vi "[ce] Create menu at runtime.vi"(4 "enable tracking (T)":bool=TRUE, 6 "after item tag":string, 7 "menu tag":string, 8 "error in":errorcluster, 9 "operation (replace)":T1(ring)=enum."replace existing menu", 10 "menu descriptor":string, 11 "menu":refnum<k9>) -> (0 "error out":errorcluster, 3 "dup menu":refnum<k9>)   [LabVIEW 2021]
doc: "The VI takes a menu descriptor and creates new menu on base of it. It can also insert or replace submenu(s) in an existing menu.\n\n<B>menu tag</B> specifies a submenu where new submenu(s) are inserted. An empty string specifies menubar. \n\n<B>after item tag</B> specifies the position where new submenu(s) are inserted. It is only used if <B>operation</B> is <insert into existing menu>. An empty string specifies the beginning of the existing submenu.\n\n<B>operation</B> specifies one of the following operations:\n <insert into existing menu> inserts the new submenu(s) to <B>menu tag</B> submenu at <B>after item tag</B> position.\n <append to existing submenu> appends the new submenu(s) to the end of <B>menu tag</B> submenu.\n <replace existing menu> replaces all the items in the <B>menu tag</B> submenu with the new submenu(s).\n\n<B>menu descriptor</B> is a multi-line string where each line contains a menu item attributes. Empty lines and lines beginning with semicolon (;) are ignored. A line starting with a dash sign (-) forms a separator in menu. A descriptor line has the following format:\n\n [SubMenuSign] ItemName : ItemTag [ : ItemParams [ : comments] ]\n\nSybMenuSign is optional parameter that can be either greater-than sign (>) marking the beginning of new submenu or less-than sign (<) marking the end of submenu. If a line begins with less-than sign (<), the rest of the line is ignored. You can form nested submenus providing that each '>' block is terminated with '<'.\n\nItemName and ItemTag are respectively a name of menu item and a tag of menu item. If an item name includes a underscore sign (_), the following character is used for ALT navigation. \n\nItemParams can contain optional specificators of the menu item separated by spaces. The specificators are not case-sensitive. You can use the following specificators:\nDIS - menu item is disabled\nCHK - menu item is checked\nKEY=CHAR - specifies a shortcut keys combination. If CHAR begins with '@' sign, the shortcut is CTRL-SHIFT-CHAR; otherwise, it is CTRL-CHAR.\n\n<B>Example:</B>\n------------\n; File menu\n> File : file\n _Open... : open : key=O\n _Close... : close : key=C\n - ;separator\n ; nested submenu\n > Configuration : config\n Parameter 1 : cfg_1 : CHK : checked\n Parameter 2 : cfg_2 : DIS : disabled\n <\n - ;separator\n E_xit : exit : key=X\n<\n; Mode menu\n> Mode : mode\nmode 1 : mode1 : KEY=@A CHK\nmode 2 : mode2 : KEY=@B DIS\nmode 3 : mode3 : KEY=@C\n<\n\n::: CalcExpress Toolkit :::\nCopyright (c) 2000-2026 Konstantin Shifershteyn. All rights reserved."
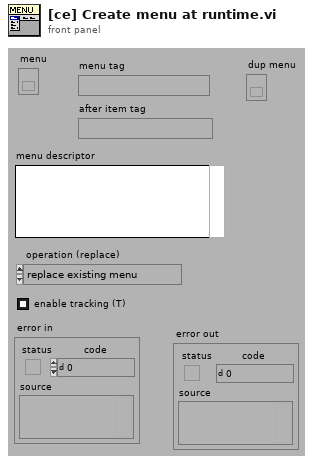
[diagram p1: front panel]
types:
  T1 = enum16{"insert into existing menu", "append to existing menu", "replace existing menu"}
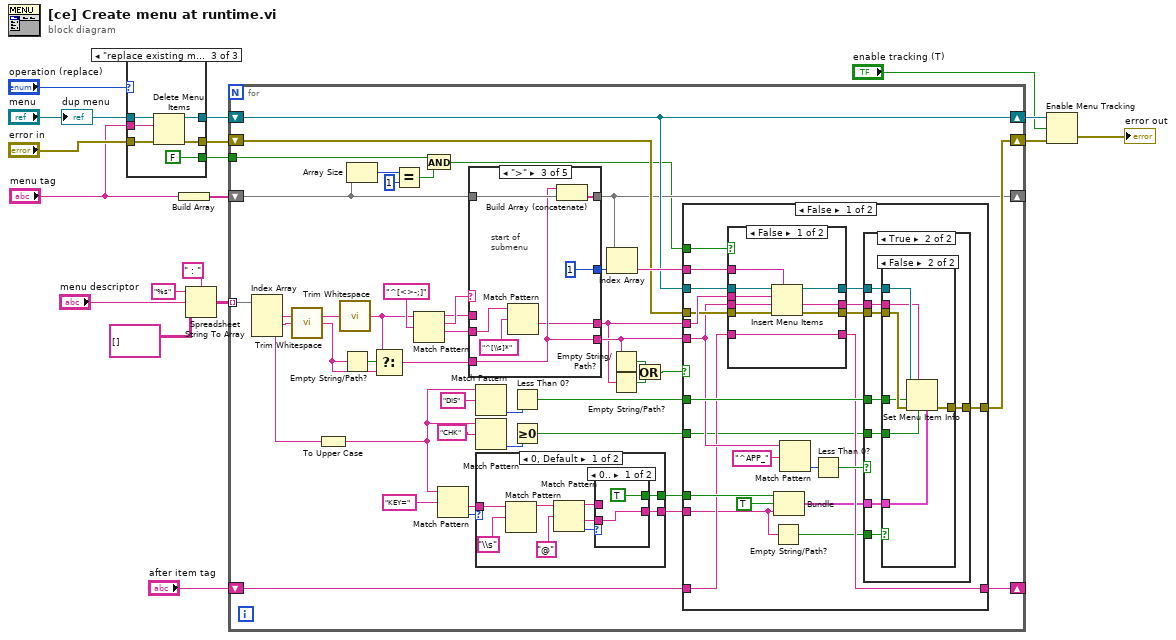
[diagram p0: block diagram]
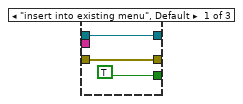
[diagram p2: hidden frame]
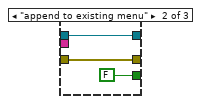
[diagram p3: hidden frame]
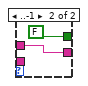
[diagram p4: hidden frame]
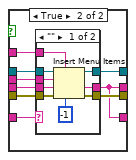
[diagram p6: hidden frame]
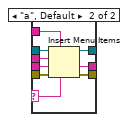
[diagram p7: hidden frame]
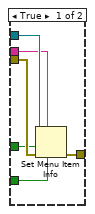
[diagram p9: hidden frame]
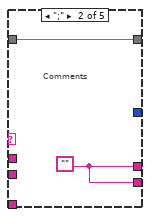
[diagram p12: hidden frame]
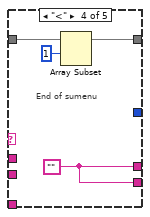
[diagram p13: hidden frame]
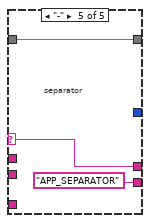
[diagram p14: hidden frame]
diagram:
  n1 = case shown="\"replace existing menu\"" "operation (replace)" {
    tunnel: [w21 w24 w30] -> w14
    tunnel: "menu" -> [w21 w24 w29]
    tunnel: [w20 w23 w28] -> w13
    tunnel: "error in" -> [w20 w23 w27]
    tunnel: [TRUE FALSE FALSE] -> w4
    tunnel: "menu tag" -> [_ _ w25]
    frame "insert into existing menu", Default {
    }
    frame "append to existing menu" {
    }
    frame "replace existing menu" {
      n2 = Delete Menu Items(6:w27, 8:w25, 9:w29) -> (0:w28:errorcluster, 3:w30:refnum<k9>)  [unwired: 1 in]
    }
  }
  n3 = Build Array("menu tag") -> (w11:string[])
  n4 = Spreadsheet String To Array(delimiter (Tab)=" : ", format string="%s", spreadsheet string="menu descriptor", array type (2D Dbl)=string[][] []) -> (array=w10:string[][])
  n5 = for {
    shift-right: [w43] -> _
    shift-left: w11 -> [w42]
    tunnel: w10 -> [w63] mode=indexing
    shift-right: [w46] -> w9
    shift-left: w14 -> [w46]
    shift-right: [w49] -> w8
    shift-left: w13 -> [w50]
    shift-right: [w48] -> _
    shift-left: "after item tag" -> [w47]
    tunnel: w4 -> [w41]
    n6 = Index Array(array=w63) -> (element #1=w33:string, element #2=w36:string, element #3=w38:string)  [unwired: 3 in]
    n7 = call <vilib>:"Trim Whitespace.vi"("string"=w36) -> ("trimmed string"=w32:string)  [unwired: 1 in]
    n8 = To Upper Case(1:w38) -> (0:w55:string)
    n9 = call <vilib>:"Trim Whitespace.vi"("string"=w33) -> ("trimmed string"=w31:string)  [unwired: 1 in]
    n10 = Empty String/Path?(string/path=w32) -> (empty?=w37:bool)
    n11 = Array Size(array=w42) -> (size(s)=w45:i32)
    n12 = Select(t=w31, s=w37, f=w32) -> (s? t:f=w35:string)
    n13 = Equal?(x=w45, y=1) -> (x = y?=w40:bool)
    n14 = Match Pattern(string=w31, regular expression="^[<>-;]") -> (before substring=w71:string, match substring=w72:string, after substring=w34:string)  [unwired: 1 in, 1 out]
    n15 = And(x=w41, y=w40) -> (x .and. y?=w39:bool)
    n16 = Match Pattern(string=w55, regular expression="KEY=") -> (after substring=w62:string, offset past match=w61:i32)  [unwired: 1 in, 2 out]
    n17 = case shown="\">\"" w72 {
      selector: w72 -> [_ _ _ _ w187]
      tunnel: w42 -> [w171 w173 w179 w181 w185]
      tunnel: w34 -> [_ _ w175 _ _]
      tunnel: [w171 w173 w180 w183 w185] -> w43
      tunnel: [w170 w172 w174 w182 w187] -> w69
      tunnel: w71 -> [w170 _ _ _ _]
      tunnel: [w169 w172 w176 w182 "APP_SEPARATOR"] -> w70
      tunnel: [_ _ 1 _ _] -> w64
      tunnel: w35 -> [w169 _ w176 _ _]
      frame "", Default {
      }
      frame ";" {
        w172 = ""
        # "Comments"
      }
      frame ">" {
        # "start of\nsubmenu"
        n18 = Match Pattern(string=w175, regular expression="^[\\s]*") -> (after substring=w174:string)  [unwired: 1 in, 3 out]
        n19 = Build Array (concatenate)(w176, w179) -> (w180:string[])
      }
      frame "<" {
        w182 = ""
        # "End of sumenu"
        n20 = Array Subset(array=w181, index=1) -> (w183:string[])  [unwired: 1 in]
      }
      frame "-" {
        # "separator"
      }
    }
    n21 = Match Pattern(string=w55, regular expression="DIS") -> (offset past match=w57:i32)  [unwired: 1 in, 3 out]
    n22 = Match Pattern(string=w55, regular expression="CHK") -> (offset past match=w59:i32)  [unwired: 1 in, 3 out]
    n23 = case shown="0, Default" w61 {
      tunnel: w62 -> [w82 _]
      tunnel: [w75 _] -> w52
      tunnel: [w74 _] -> w51
      frame 0, Default {
        n24 = Match Pattern(string=w82, regular expression="\\s") -> (before substring=w79:string)  [unwired: 1 in, 3 out]
        n25 = Match Pattern(string=w79, regular expression="@") -> (before substring=w77:string, after substring=w76:string, offset past match=w78:i32)  [unwired: 1 in, 1 out]
        n26 = case shown="0.." w78 {
          tunnel: [w84 w86] -> w74
          tunnel: w77 -> [_ w86]
          tunnel: [TRUE FALSE] -> w75
          tunnel: w76 -> [w84 _]
          frame 0.. {
          }
          frame ..-1 {
          }
        }
      }
      frame ..-1 {
      }
    }
    n27 = Less Than 0?(x=w57) -> (x < 0?=w53:bool)
    n28 = Greater Or Equal To 0?(x=w59) -> (x >= 0?=w54:bool)
    n29 = Index Array(array=w43, index=w64) -> (element=w65:string)
    n30 = Empty String/Path?(string/path=w70) -> (empty?=w68:bool)
    n31 = Empty String/Path?(string/path=w69) -> (empty?=w67:bool)
    n32 = Or(x=w68, y=w67) -> (x .or. y?=w66:bool)
    n33 = case shown="False" w66 {
      tunnel: w69 -> [w105 _]
      tunnel: w70 -> [w97 _]
      tunnel: w65 -> [w95 _]
      tunnel: w46 -> [w108 _]
      tunnel: w50 -> [w103 w168]
      tunnel: [w102 w168] -> w49
      tunnel: w54 -> [w92 _]
      tunnel: w53 -> [w101 _]
      tunnel: w52 -> [w100 _]
      tunnel: w51 -> [w87 _]
      tunnel: w47 -> [w94 w167]
      tunnel: [w93 w167] -> w48
      tunnel: w39 -> [w90 _]
      frame False {
        n34 = case shown="False" w90 {
          tunnel: w108 -> [w117 w126]
          tunnel: [w116 w125] -> w107
          tunnel: [w115 w124] -> w106
          tunnel: w105 -> [w114 w123]
          tunnel: [w113 w118] -> w104
          tunnel: w103 -> [w112 w122]
          tunnel: w97 -> [w111 w119]
          tunnel: w95 -> [w110 w120]
          tunnel: w94 -> [w109 w121]
          tunnel: [w109 w118] -> w93
          frame False {
            n35 = Insert Menu Items(5:w110, 6:w112, 7:w111, 8:w114, 9:w117) -> (0:w115:errorcluster, 1:w113:string, 3:w116:refnum<k9>)  [unwired: 1 in]
          }
          frame True {
            n36 = case shown="\"\"" w121 {
              selector: w121 -> [_ w136]
              tunnel: w126 -> [w135 w144]
              tunnel: [w134 w143] -> w125
              tunnel: [w133 w142] -> w124
              tunnel: w123 -> [w132 w141]
              tunnel: [w131 w140] -> w118
              tunnel: w122 -> [w130 w139]
              tunnel: w119 -> [w129 w138]
              tunnel: w120 -> [w128 w137]
              frame "" {
                n37 = Insert Menu Items(4:-1, 5:w128, 6:w130, 7:w129, 8:w132, 9:w135) -> (0:w133:errorcluster, 1:w131:string, 3:w134:refnum<k9>)
              }
              frame "a", Default {
                n38 = Insert Menu Items(4:w136, 5:w137, 6:w139, 7:w138, 8:w141, 9:w144) -> (0:w142:errorcluster, 1:w140:string, 3:w143:refnum<k9>)
              }
            }
          }
        }
        n39 = Empty String/Path?(string/path=w87) -> (empty?=w88:bool)
        n40 = Bundle(w100, TRUE, w87) -> (w91:cluster{bool, bool, string})  [unwired: 1 in]
        n41 = Match Pattern(string=w97, regular expression="^APP_") -> (offset past match=w98:i32)  [unwired: 1 in, 3 out]
        n42 = Less Than 0?(x=w98) -> (x < 0?=w96:bool)
        n43 = case shown="True" w96 {
          tunnel: w107 -> [_ w153]
          tunnel: w106 -> [w145 w152]
          tunnel: w104 -> [_ w151]
          tunnel: [w145 w150] -> w102
          tunnel: w101 -> [_ w149]
          tunnel: w92 -> [_ w148]
          tunnel: w91 -> [_ w147]
          tunnel: w88 -> [_ w146]
          frame False {
          }
          frame True {
            n44 = case shown="False" w146 {
              tunnel: w153 -> [w159 w166]
              tunnel: w152 -> [w158 w165]
              tunnel: w151 -> [w157 w164]
              tunnel: [w156 w163] -> w150
              tunnel: w149 -> [w155 w162]
              tunnel: w148 -> [w154 w161]
              tunnel: w147 -> [_ w160]
              frame True {
                n45 = Set Menu Item Info(6:w154, 7:w157, 8:w158, 9:w155, 11:w159) -> (0:w156:errorcluster)  [unwired: 2 in, 1 out]
              }
              frame False {
                n46 = Set Menu Item Info(4:w160, 6:w161, 7:w164, 8:w165, 9:w162, 11:w166) -> (0:w163:errorcluster)  [unwired: 1 in, 1 out]
              }
            }
          }
        }
      }
      frame True {
      }
    }
  }
  n47 = Enable Menu Tracking(2:w8, 3:"enable tracking (T)", 4:w9) -> (0:→"error out":errorcluster)  [unwired: 1 out]
  "dup menu" <- "menu"
